vi "Remove_User_in_program.vi"(8 "error in (no error)":errorcluster) -> (0 "error out":errorcluster)   [LabVIEW 2021]
uses:
  Option control.ctl
panel:
  in  "Tab Control":enum32{"Page 2"}(tab)
  in  "LOG ID":string
  in  "OK":bool caption="OK2"
  in  "PASSWORD":string
  # "Enter opertor Name and ID\n and press OK"
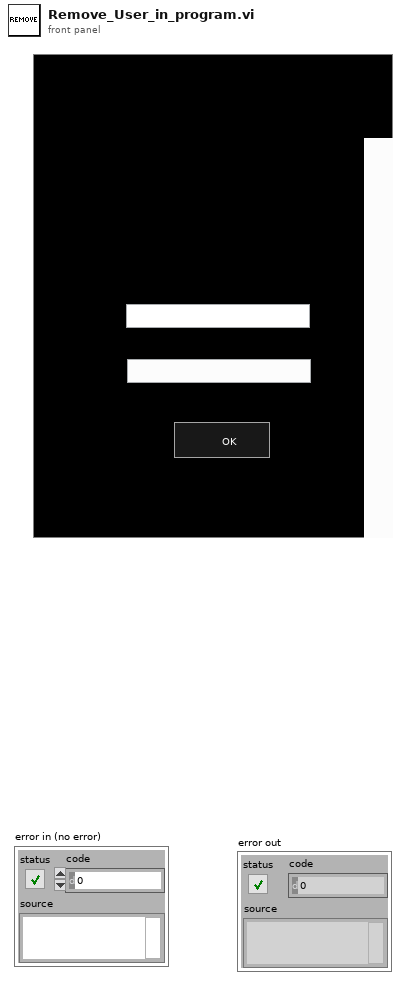
[diagram p1: front panel]
types:
  T1 = typedef "Option control.ctl" = enum16{"Input", "Output"}
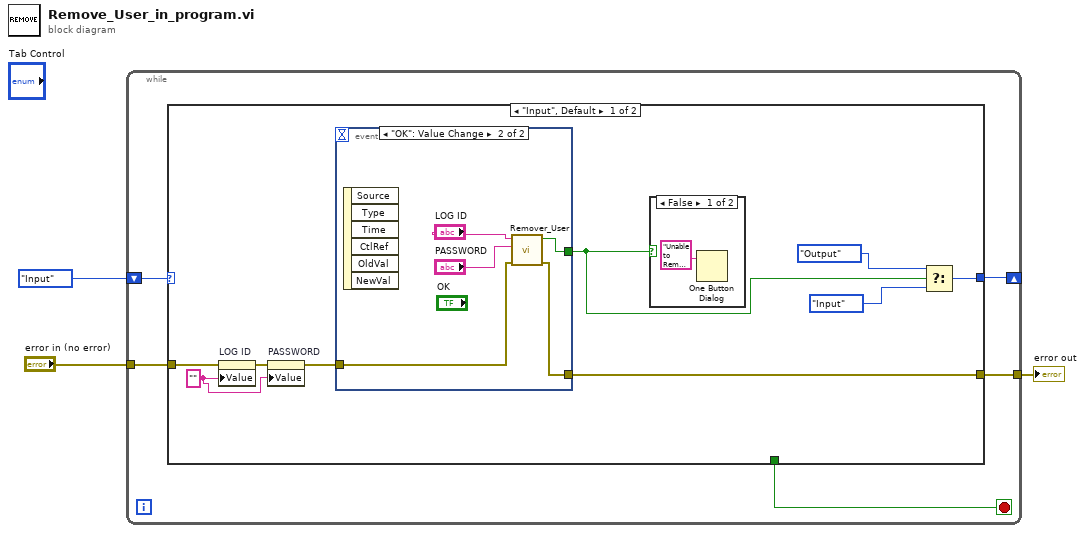
[diagram p0: block diagram]
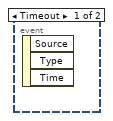
[diagram p3: hidden frame]
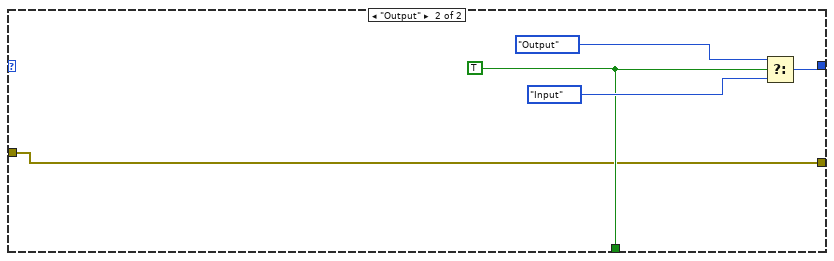
[diagram p4: hidden frame]
diagram:
  n1 = while {
    shift-right: [w7] -> _
    shift-left: Option_control."Input" -> [w8]
    tunnel: "error in (no error)" -> [w5]
    tunnel: [w4] -> w1
    stop <- w6 stop-if-true
    n2 = case shown="\"Input\", Default" w8 {
      tunnel: [w15 w26] -> w7
      tunnel: [_ w25] -> w6
      tunnel: w5 -> [w11 w24]
      tunnel: [w13 w24] -> w4
      frame "Input", Default {
        w9 = "" ("LOG ID")
        n3 = property on="LOG ID" class="Str"(error in=w11, "Value"=w9) -> (error out=w12:errorcluster)  [unwired: 1 in, 1 out]
        n4 = property on="PASSWORD" class="Str"(error in=w12, "Value"=w9) -> (error out=w10:errorcluster)  [unwired: 1 in, 1 out]
        n5 = event shown="[1] \"OK\": Value Change" {
          selector: _ -> [_ _]
          dyn-events: _ -> [_ _]
          timeout: _ -> [_ _]
          tunnel: [_ w23] -> w14
          tunnel: w10 -> [_ w21]
          tunnel: [_ w22] -> w13
          event Timeout {
            n6 = event-data() -> ()  [unwired: 1 in, 3 out]
          }
          event "OK": Value Change {
            n7 = event-data() -> ()  [unwired: 1 in, 6 out]
            n8 = call "Remover_User.vi"("error in (no error)"=w21, "Password"="PASSWORD", "Name"="LOG ID") -> ("error out"=w22:errorcluster, "Result"=w23:bool)  [unwired: 7 in]
          }
        }
        n9 = case shown="False" w14 {
          frame False {
            n10 = One Button Dialog(message="Unable to Remove a user") -> ()  [unwired: 1 in, 1 out]
          }
          frame True {
          }
        }
        n11 = Select(t=Option_control."Output", s=w14, f=Option_control."Input") -> (s? t:f=w15:T1)
      }
      frame "Output" {
        w25 = TRUE ("s")
        n12 = Select(t=Option_control."Output", s=w25, f=Option_control."Input") -> (s? t:f=w26:T1)
      }
    }
  }
  "error out" <- w1
